vi "Write Module Page Property.vi"(8 "error in (no error)":errorcluster, 10 "RSI Module":refnum<class "RSI Module.lvclass">, 11 "Node Ptr In":T1 format="%.0x") -> (0 "error out":errorcluster, 2 "RSI Module out":refnum<class "RSI Module.lvclass">, 3 "Node Ptr Out":T1 format="%.0x")   [LabVIEW 2020, in "Modules.lvlib" / "RSI Module.lvclass"]
uses:
  RSI Module.lvclass
  <vilib>/NI VeriStand/Custom Device API/Custom Device Item Ref.ctl
  Debug.vi
  Class Property Strings.vi
  <vilib>/NI VeriStand/Custom Device API/Set Item Property (String).vi
  <vilib>/NI VeriStand/Custom Device API/Custom Device API.lvlib
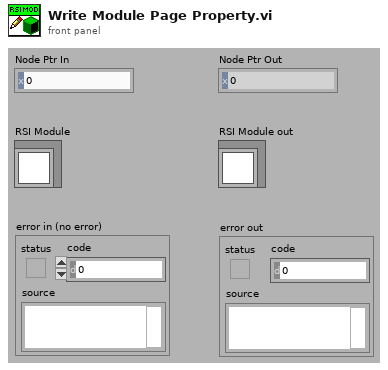
[diagram p1: front panel]
types:
  T1 = typedef "Custom Device API.lvlib/Custom Device Item Ref.ctl" = u64
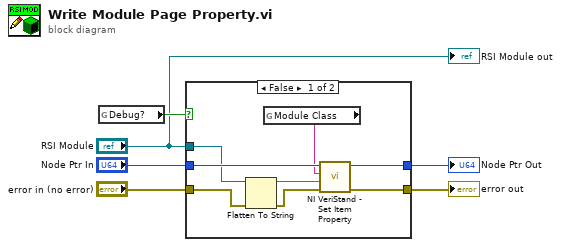
[diagram p0: block diagram]
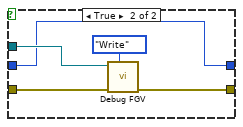
[diagram p2: hidden frame]
diagram:
  n1 = global read "Debug.vi" "Debug?"() -> (w2:bool)
  n2 = case shown="False" w2 {
    tunnel: "Node Ptr In" -> [w14 w15]
    tunnel: [w13 w15] -> w5
    tunnel: [w12 w16] -> w4
    tunnel: "RSI Module" -> [w7 w17]
    tunnel: "error in (no error)" -> [w10 w18]
    frame False {
      n3 = Flatten To String(anything=w7, error in (no error)=w10) -> (data string=w11:string, error out=w9:errorcluster)  [unwired: 2 in, 1 out]
      n4 = global read "Class Property Strings.vi" "Module Class"() -> (w8:string)
      n5 = call-poly <vilib>:"NI VeriStand - Set Item Property.vi"("error in (no error)"=w9, "Value"=w11, "Property Name"=w8, "Item Ref in"=w14) -> ("error out"=w12:errorcluster, "Item Ref out"=w13:T1)  [unwired: 5 in, 1 out]
    }
    frame True {
      n6 = call "Debug FGV.vi"("Action"=enum16{"Read", "Write"}."Write", "error in (no error)"=w18, "RSI Module in"=w17) -> ("error out"=w16:errorcluster)  [unwired: 7 in, 1 out]
    }
  }
  "Node Ptr Out" <- w5
  "error out" <- w4
  "RSI Module out" <- "RSI Module"
